vi "Report.vi"(10 "Array 2":string[][](array[string])=[["dsfds", "-797", "-798", "-1.00", "No Alarm", "<", "12"]], 11 "text data":string[][](array[string])) -> ()   [LabVIEW 2024]
uses:
  <vilib>/Utility/NIReport.llb/Word/NI_Word.lvclass
  <vilib>/addons/_office/NI_ReportGenerationToolkit.lvlib
  <vilib>/Utility/NIReport.llb/NI_report.lvclass
  <vilib>/Utility/NIReport.llb/Report Type.ctl
  <vilib>/Utility/NIReport.llb/NI_ReportGenerationCore.lvlib
  <vilib>/addons/_office/_exclsub.llb/font.ctl
  <vilib>/Utility/NIReport.llb/Append Image to Report (path wrap).vi
  <vilib>/Utility/NIReport.llb/Append Text Table to Report (wrap).vi
  <vilib>/Utility/NIReport.llb/image depth.ctl
  Wave forms.vi
  Global 1.vi
  <vilib>/Utility/NIReport.llb/HTML Report Image Alignment.ctl
panel:
  in  "MS Office parameters":T1
  in  "alignment (default) 2":T2
  out "Waveform Graph":dbl[](graph)
  in  "numerical data":dbl[][](array[numeric]) format="%.2f"
  in  "error in (no error)":errorcluster
  in  "font settings source":u16(ring) items=["VI Inputs", "Font Dialog Box"]
  in  "alignment (default)":T2
  in  "path or URL of image":path
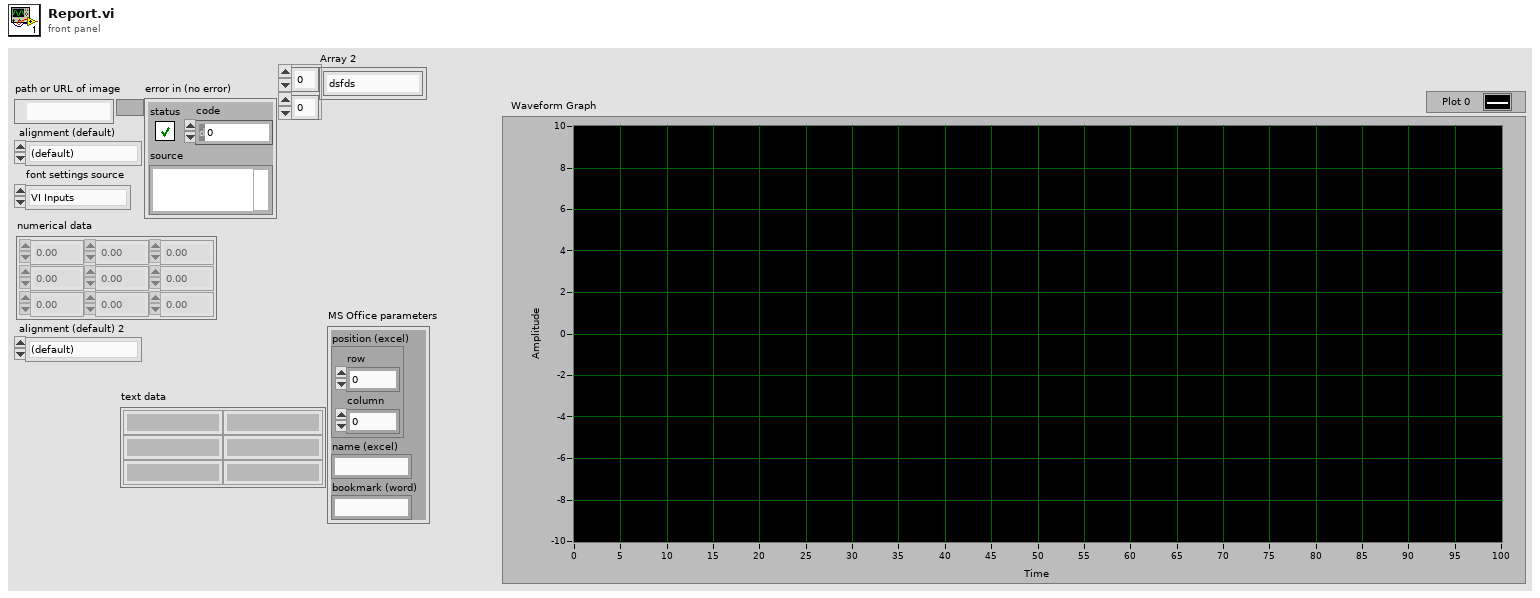
[diagram p1: front panel]
types:
  T1 = cluster{"position (excel)":cluster{"row":i32, "column":i32}, "name (excel)":string, "bookmark (word)":string}
  T2 = typedef "NI_ReportGenerationCore.lvlib/HTML Report Image Alignment.ctl" = enum16{"(default)", "LEFT", "RIGHT", "TOP", "TEXTTOP", "MIDDLE", "ABSMIDDLE", "BASELINE", "BOTTOM", "ABSBOTTOM"}
  T3 = cluster{"Charset (-1)":i16, "Weight (-1)":i16, "Name":string, "Size":string}
  T4 = typedef "NI_ReportGenerationToolkit.lvlib/font.ctl" = cluster{"font name":string, "font size":dbl, "bold":u16, "italic":u16, "underline":u16, "strike through":u16, "font color":u32}
  T5 = cluster{"Italic":enum16{"Italic Unchanged", "Italic On", "Italic Off"}, "Strike Through":enum16{"Strike Through Unchanged", "Strike Through On", "Strike Through Off"}, "Underline":enum16{"Underline Unchanged", "Underline On", "Underline Off"}, "Bold":enum16{"Bold Unchanged", "Bold On", "Bold Off"}}
  T6 = typedef "NI_ReportGenerationCore.lvlib/Report Type.ctl" = enum16{"HTML", "Word", "Excel"}
  T7 = typedef "NI_ReportGenerationCore.lvlib/image depth.ctl" = u16
  T8 = cluster{"OutsideLineStyle":i32, "OutsideColor":i32, "OutsideLineWidth":i32, "InsideLineStyle":i32, "InsideColor":i32, "InsideLineWidth":i32, "BackgroundPatternColor":i32}
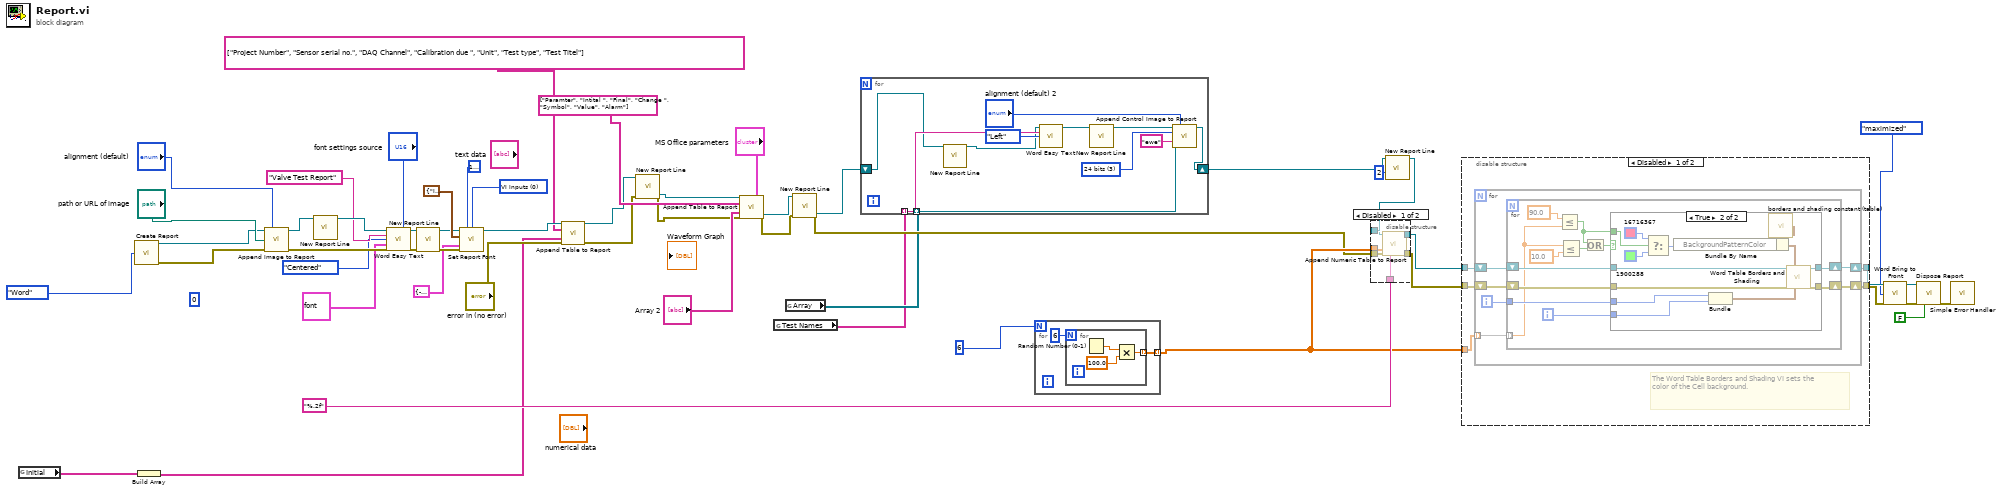
[diagram p0: block diagram]
diagram:
  w1 = u16 0 items=["VI Inputs", "Font Dialog Box"] ("font settings source (VI Inputs)")
  (unwired) 0 ("start (-1)")
  n1 = global read "Global 1.vi" "Initial"() -> (w8:string[])
  n2 = call <vilib>:"Create Report.vi"("report type"=Report_Type."Word" ("Report Type")) -> ("report out"=w3:refnum<class "NI_report.lvclass">, "error out"=w40:errorcluster)  [unwired: 13 in]
  n3 = Build Array(w8) -> (w7:string[][])
  n4 = call-poly <vilib>:"Append Image to Report.vi"("report in"=w3, "alignment (default)"="alignment (default)", "path or URL of image"="path or URL of image", "error in (no error)"=w40) -> ("report out"=w35:refnum<class "NI_report.lvclass">, "error out"=w34:errorcluster)  [unwired: 8 in, 2 out]
  n5 = call-dynamic "New Report Line.vi"("report in"=w35) -> ("report out"=w31:refnum<class "NI_report.lvclass">)  [unwired: 13 in, 1 out]
  n6 = call <vilib>:"Word Easy Text.vi"("report in"=w31, "font settings source"="font settings source", "text"="Valve Test Report", "alignment (left)"=enum16{"Left", "Centered", "Right", "Justify"}."Centered", "font"=T4 {"font name"="Times New Roman", "font size"=0.0, "bold"=1, "italic"=0, "underline"=1, "strike through"=0, "font color"=16777216}, "error in (no error)"=w34) -> ("report out"=w32:refnum<class "NI_report.lvclass">, "error out"=w33:errorcluster)  [unwired: 7 in, 1 out]
  n7 = call-dynamic "New Report Line.vi"("report in"=w32, "error in (no error)"=w33) -> ("report out"=w37:refnum<class "NI_report.lvclass">, "error out"=w36:errorcluster)  [unwired: 12 in]
  n8 = call-dynamic "Set Report Font.vi"("report in"=w37, "text color (unchanged)"=u32 16777216, "font settings source (VI Inputs)"=w1, "text options"=T5 {"Italic"=enum."Italic Unchanged", "Strike Through"=enum."Strike Through Unchanged", "Underline"=enum."Underline Unchanged", "Bold"=enum."Bold On"}, "font settings"=T3 {"Charset (-1)"=-1, "Weight (-1)"=-1, "Name"="", "Size"=" "}, "error in (no error)"=w36) -> ("report out"=w26:refnum<class "NI_report.lvclass">)  [unwired: 7 in, 2 out]
  n9 = call-poly <vilib>:"Append Table to Report.vi"("report in"=w26, "column headers"=string[] ["Project Number", "Sensor serial no.", "DAQ Channel", "Calibration due ", "Unit", "Test type", "Test Titel"], "text data"=w7, "error in (no error)"="error in (no error)") -> ("report out"=w18:refnum<class "NI_report.lvclass">, "error out"=w16:errorcluster)  [unwired: 8 in, 2 out]
  n10 = call-dynamic "New Report Line.vi"("report in"=w18, "error in (no error)"=w16) -> ("report out"=w17:refnum<class "NI_report.lvclass">, "error out"=w15:errorcluster)  [unwired: 12 in]
  n11 = call-poly <vilib>:"Append Table to Report.vi"("report in"=w17, "MS Office parameters"="MS Office parameters", "column headers"=string[] ["Paramter", "Intital ", "Final", "Change ", "Symbol", "Value", "Alarm"], "text data"="Array 2", "error in (no error)"=w15) -> ("report out"=w22:refnum<class "NI_report.lvclass">, "error out"=w21:errorcluster)  [unwired: 7 in, 2 out]
  n12 = global read "Wave forms.vi" "Test Names"() -> (w6:string[])
  n13 = global read "Wave forms.vi" "Array"() -> (w10:refnum<vi>[])
  n14 = call-dynamic "New Report Line.vi"("report in"=w22, "error in (no error)"=w21) -> ("report out"=w14:refnum<class "NI_report.lvclass">, "error out"=w23:errorcluster)  [unwired: 12 in]
  n15 = for {
    shift-right: [w64] -> w13
    shift-left: w14 -> [w55]
    tunnel: w10 -> [w60] mode=indexing
    tunnel: w6 -> [w59] mode=indexing
    w63 = T7 3 items=["B&W", "4 bits", "8 bits", "24 bits"] ("image depth")
    n16 = call-dynamic "New Report Line.vi"("report in"=w55) -> ("report out"=w54:refnum<class "NI_report.lvclass">)  [unwired: 13 in, 1 out]
    n17 = call <vilib>:"Word Easy Text.vi"("report in"=w54, "text"=w59, "alignment (left)"=enum16{"Left", "Centered", "Right", "Justify"}."Left") -> ("report out"=w57:refnum<class "NI_report.lvclass">)  [unwired: 10 in, 2 out]
    n18 = call-dynamic "New Report Line.vi"("report in"=w57) -> ("report out"=w56:refnum<class "NI_report.lvclass">)  [unwired: 13 in, 1 out]
    n19 = call-dynamic "Append Control Image to Report.vi"("report in"=w56, "alignment (default)"="alignment (default) 2", "image depth"=w63, "ctrl reference"=w60, "description"="ewe") -> ("report out"=w64:refnum<class "NI_report.lvclass">)  [unwired: 7 in, 3 out]
  }
  n20 = for {
    N: 6 -> [_]
    tunnel: [w65] -> w42 mode=indexing
    n21 = for {
      N: 6 ("dimension size") -> [_]
      tunnel: [w67] -> w65 mode=indexing
      n22 = Random Number (0-1)() -> (number: 0 to 1=w69:dbl)
      n23 = Multiply(x=w69, y=100.0) -> (x*y=w67:dbl)
    }
  }
  n24 = call-dynamic "New Report Line.vi"("report in"=w13, "number of lines (1)"=2) -> ("report out"=w12:refnum<class "NI_report.lvclass">)  [unwired: 12 in, 1 out]
  n25 = disable-structure shown="Disabled" {
    disable-tunnel: [w75 w77] -> w53
    disable-tunnel: [w74 w76] -> w52
    disable-tunnel: "%.2f" ("format string") -> [w73 _]
    disable-tunnel: w42 -> [w72 _]
    disable-tunnel: w23 -> [w71 w76]
    disable-tunnel: w12 -> [w70 w77]
    frame Disabled {
      n26 = call-dynamic "Append Numeric Table to Report.vi"("report in"=w70, "numerical data"=w72, "error in (no error)"=w71, "format string (%.3f)"=w73) -> ("report out"=w75:refnum<class "NI_report.lvclass">, "error out"=w74:errorcluster)  [unwired: 8 in, 2 out]
    }
    frame Enabled {
    }
  }
  n27 = disable-structure shown="Disabled" {
    disable-tunnel: w53 -> [w82 w116]
    disable-tunnel: w52 -> [w81 w117]
    disable-tunnel: [w80 w117] -> w49
    disable-tunnel: [w79 w116] -> w48
    disable-tunnel: w42 -> [w78 _]
    frame Disabled {
      # "The Word Table Borders and Shading VI sets the color of the Cell background."
      n28 = for {
        shift-right: [w87] -> w79
        shift-left: w82 -> [w88]
        shift-right: [w85] -> w80
        shift-left: w81 -> [w86]
        tunnel: w78 -> [w83] mode=indexing
        i -> [w84]
        n29 = for {
          shift-right: [w99] -> w87
          shift-left: w88 -> [w98]
          shift-right: [w100] -> w85
          shift-left: w86 -> [w97]
          tunnel: w84 -> [w95]
          tunnel: w83 -> [w93] mode=indexing
          i -> [w89]
          n30 = Less Or Equal?(x=90.0 ("y"), y=w93) -> (x <= y?=w92:bool)
          n31 = Less Or Equal?(x=w93, y=10.0) -> (x <= y?=w91:bool)
          n32 = Or(x=w92, y=w91) -> (x .or. y?=w90:bool)
          n33 = case shown="True" w90 {
            tunnel: [w101 w115] -> w100
            tunnel: [w102 w114] -> w99
            tunnel: w89 -> [_ w103]
            tunnel: w95 -> [_ w104]
            tunnel: w98 -> [w102 w107]
            tunnel: w97 -> [w101 w106]
            tunnel: w92 -> [_ w105]
            frame False {
            }
            frame True {
              n34 = Select(t=u32 16716367, s=w105, f=u32 1900288) -> (s? t:f=w108:u32)
              n35 = Bundle(w104, w103) -> (w111:cluster{i32, i32})  [unwired: 1 in]
              n36 = call <vilib>:"borders and shading constant (table).vi"() -> ("borders and shading"=w113:T8)
              n37 = Bundle By Name(cluster=w113, "BackgroundPatternColor"=w108) -> (w112:T8)
              n38 = call <vilib>:"Word Table Borders and Shading.vi"("report in"=w107, "borders and shading"=w112, "error in (no error)"=w106, "start (-1, -1)"=w111) -> ("report out"=w114:refnum<class "NI_report.lvclass">, "error out"=w115:errorcluster)  [unwired: 10 in]
            }
          }
        }
      }
    }
    frame Enabled {
    }
  }
  n39 = call <vilib>:"Word Bring to Front.vi"("report in"=w48, "window state (maximized)"=enum16{"maximized", "minimized", "normal"}."maximized", "error in (no error)"=w49) -> ("report out"=w47:refnum<class "NI_report.lvclass">, "error out"=w46:errorcluster)  [unwired: 11 in]
  n40 = call-dynamic "Dispose Report.vi"("report in"=w47, "error in (no error)"=w46, "close report? (T)"=FALSE ("Close Report? (T)")) -> ("error out"=w45:errorcluster)  [unwired: 12 in]
  n41 = call <vilib>:"Simple Error Handler.vi"("error in (no error)"=w45) -> ()  [unwired: 4 in, 5 out]
